vi "MB_Master Comm Tester.vi"() -> ()   [LabVIEW 2012]
doc: "Modbus Comm Tester\n\nThis VI demonstrates the usage of the Modbus Master API for both TCP and Serial connections.\nIt is also a useful tool for testing communication with your modbus device. You can test different\ncommunication parameters and coil/register address ranges without having to write any code.\n\nCopyright (c) 2016, Plasmionique Inc.\nAll rights reserved.\n\nLicense: BSD (2-Clause) - http://opensource.org/licenses/BSD-2-Clause"
uses:
  MB_Master/MB_Master.lvclass
  MB_ADU/MB_ADU.lvclass/MB_ADU.ctl
  MB_ADU/Read TX Data.vi
  MB_ADU/Read RX Data.vi
  MB_ADU/Read RX Timestamp.vi
  MB_Master_Serial/MB_Master_Serial.lvclass
  MB Master.lvlib
  MB_ADU/MB_ADU.lvclass
  MB_Master_TCP/MB_Master_TCP.lvclass
panel:
  in  "Poll Period (ms)":i32=100
  in  "Tab Control":enum32{"Page 1", "Page 2"}(tab)
  in  "Retries":i32=1
  in  "Timeout (ms)":u32=300
  in  "Flow Control":u16(ring) items=["None", "XON/XOFF", "RTS/CTS", "XON/XOFF & RTS/CTS", "DTR/DSR", "XON/XOFF & DTR/DSR"]
  in  "Parity":u16(ring) items=["None", "Odd", "Even", "Mark", "Space"]
  in  "Stop Bits":u16(ring)=10 items=["1.0"=10, "1.5"=15, "2.0"=20]
  in  "Baud Rate (bps)":u32(ring)=19200 items=["9600"=9600, "19200"=19200, "38400"=38400, "57600"=57600, "115200"=115200, "460800"=460800, "921600"=921600]
  in  "Slave Address":u8=1
  in  "Mode":enum16{"RTU", "ASCII"}(ring)
  in  "COM Port":refnum<visa-resource-name>
  in  "TCP_Port":u16=502 caption="Port"
  in  "IP Address":string="localhost"
  in  "TCP_Timeout":i32=10000 caption="Timeout (ms)"
  in  "TCP_Slave ID":u8=255 caption="Slave ID" format="%.0x"
  in  "Type":enum16{"Serial", "TCP"}(ring) caption="Connection Type"
  out "dt (ms)":u32
  in  "DI Poll":bool
  in  "IR Poll":bool
  in  "Exit":bool
  out "Last Error Time":string
  out "Last RX Time":string
  in  "Write Hld Regs":bool
  in  "Read Hld Regs":bool
  in  "HR QTY":u16=1 caption="Quantity"
  in  "HR SA":u16 caption="Starting Address" format="%.0x"
  in  "Holding Registers":u16[](array[numeric])
  in  "Read In Regs":bool
  in  "IR QTY":u16=1 caption="Quantity"
  in  "IR SA":u16 caption="Starting Address" format="%.0x"
  out "Input Registers":u16[](array[numeric])
  in  "Read DIs":bool
  in  "DI QTY":u16=1 caption="Quantity"
  in  "DI SA":u16 caption="Starting Address" format="%.0x"
  out "Discrete Inputs":bool[](array[boolean])
  in  "Write Coils":bool
  in  "Read Coils":bool
  in  "Coil QTY":u16=1 caption="Quantity"
  in  "Coil SA":u16 caption="Starting Address" format="%.0x"
  in  "Coils":bool[](array[boolean])
  out "Last TX":string
  out "Last RX":string
  out "Last Error Status":errorcluster
  out "Open?":bool
  in  "Close":bool
  in  "Open":bool
  # "Input Registers"
  # "Discrete Inputs"
  # "Communication Settngs"
  # "Communication Status"
  # "Holding Registers"
  # "Coils"
  # "See block diagram for description and usage notes."
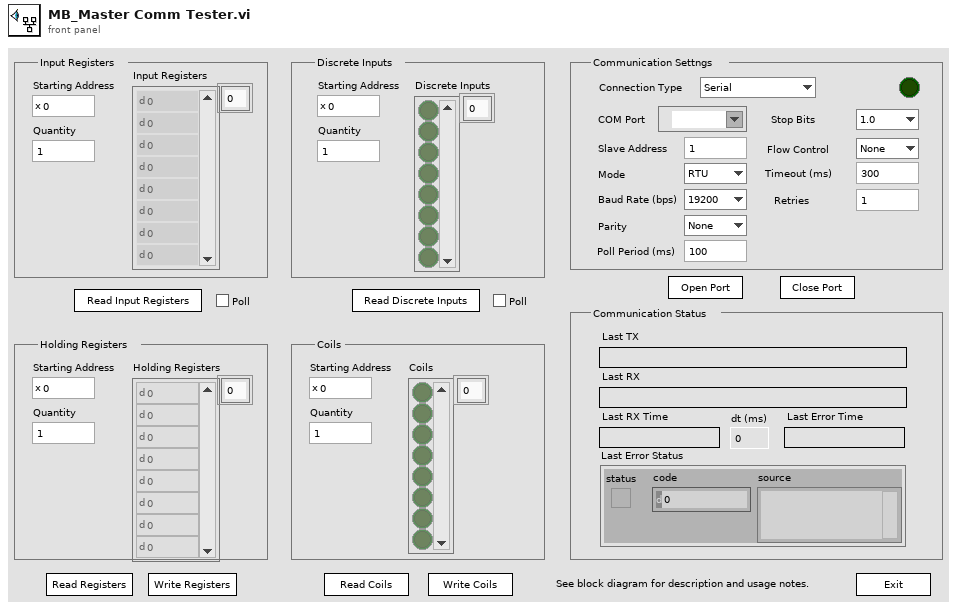
[diagram p1: front panel]
types:
  T1 = cluster{"baud rate (bps)":u32, "stop bits":u16, "parity":u16, "flow control":u16, "timeout":u32, "retries":i32}
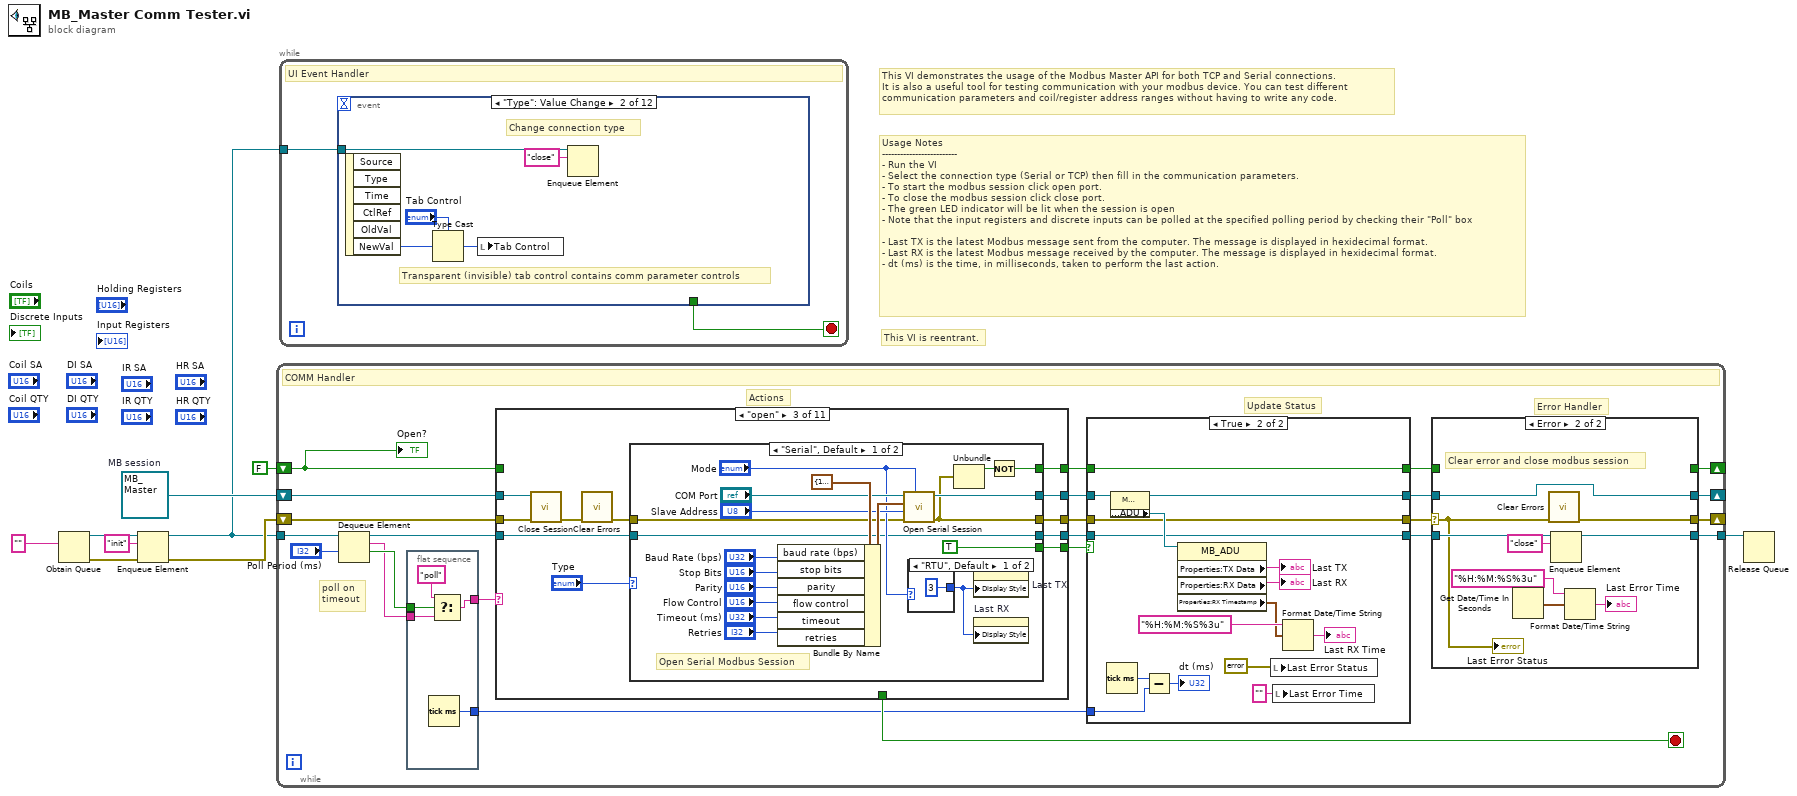
[diagram p0: block diagram]
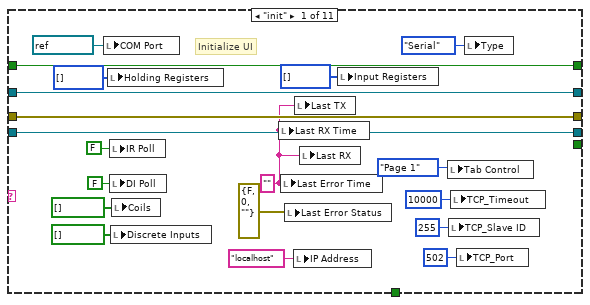
[diagram p4: hidden frame]
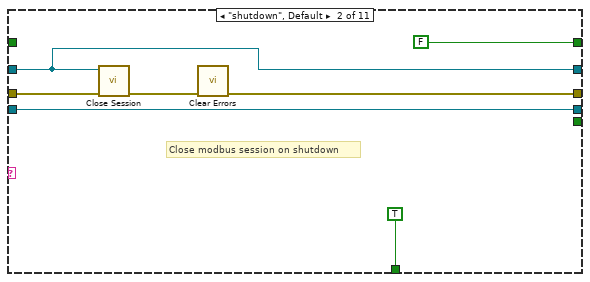
[diagram p5: hidden frame]
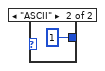
[diagram p6: hidden frame]
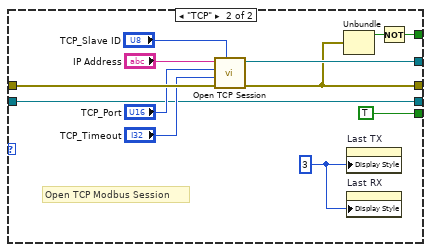
[diagram p7: hidden frame]
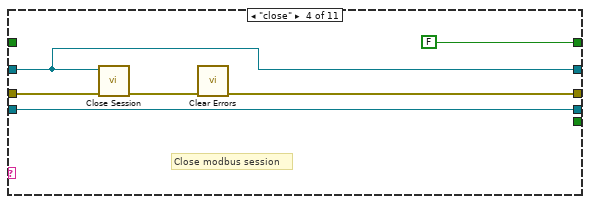
[diagram p8: hidden frame]
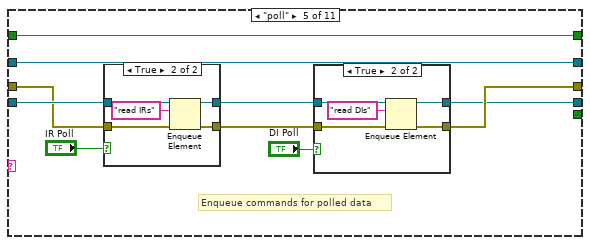
[diagram p9: hidden frame]
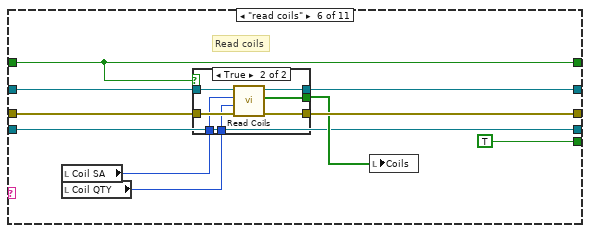
[diagram p12: hidden frame]
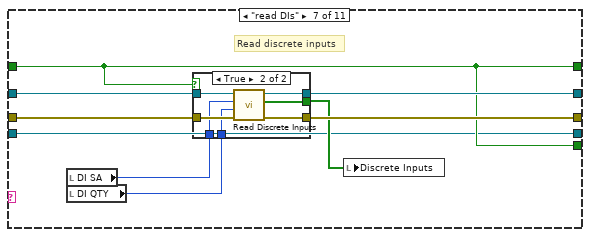
[diagram p14: hidden frame]
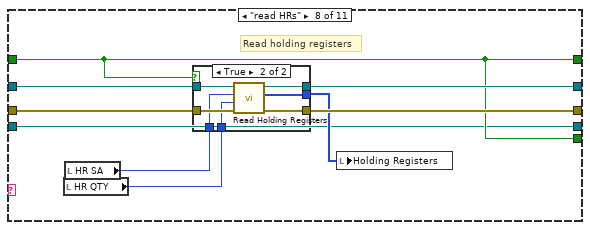
[diagram p16: hidden frame]
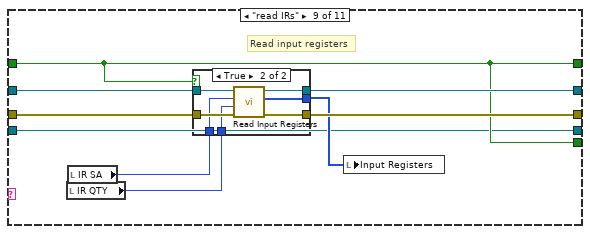
[diagram p18: hidden frame]
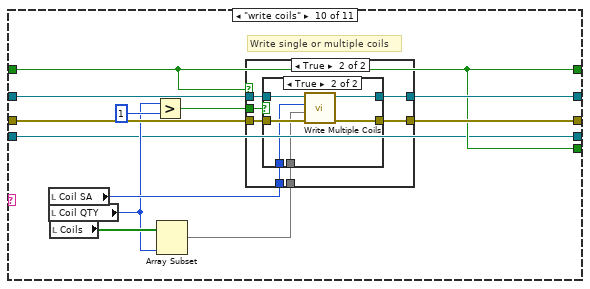
[diagram p20: hidden frame]
diagram:
  w7 = refnum<class "MB_Master.lvclass"> refnum  # MB session
  # "This VI is reentrant."
  # "Usage Notes\n-------------------------\n- Run the VI\n- Select the connection type (Serial or TCP) then fill in the communication parameters.\n- To start the modbus session click open port.\n- To close the modbus session click close port.\n- The green LED indicator will be lit when the session is open\n- Note that the input registers and discrete inputs can be polled at the specified polling period by checking their \"Poll\" box\n\n- Last TX is the latest Modbus message sent from the computer. The message is displayed in hexidecimal format.\n- Last RX is the latest Modbus message received by the computer. The message is displayed in hexidecimal format. \n- dt (ms) is the time, in milliseconds, taken to perform the last action."
  # "This VI demonstrates the usage of the Modbus Master API for both TCP and Serial connections.\nIt is also a useful tool for testing communication with your modbus device. You can test different\ncommunication parameters and coil/register address ranges without having to write any code."
  n1 = Obtain Queue(element data type="") -> (queue out=w6:refnum<queue>, error out=w4:errorcluster)  [unwired: 4 in, 1 out]
  n2 = Enqueue Element(queue=w6, element="init", error in (no error)=w4) -> (queue out=w2:refnum<queue>, error out=w3:errorcluster)  [unwired: 1 in, 1 out]
  n3 = while {
    tunnel: w2 -> [w33]
    shift-right: [w16] -> _
    shift-left: w7 -> [w32]
    shift-right: [w23] -> _
    shift-left: w3 -> [w24]
    shift-right: [w18] -> _
    shift-left: FALSE -> [w28]
    tunnel: [w22] -> w1
    stop <- w31 stop-if-true
    # "poll on\ntimeout"
    # "Actions"
    # "Error Handler"
    # "Update Status"
    # "COMM Handler"
    n4 = Dequeue Element(queue=w33, timeout in ms (-1)="Poll Period (ms)") -> (queue out=w30:refnum<queue>, element=w20:string, timed out?=w21:bool)  [unwired: 1 in, 1 out]
    n5 = flat-sequence {
      tunnel: [w51] -> w25
      tunnel: w21 -> [w50]
      tunnel: w20 -> [w49]
      tunnel: [w47] -> w19
      frame #0 {
        n6 = Tick Count (ms)() -> (millisecond timer value=w51:u32)
        n7 = Select(t="poll", s=w50, f=w49) -> (s? t:f=w47:string)
      }
    }
    n8 = case shown="\"open\"" w19 {
      tunnel: [w89 w94 w108 w144 w149 w179 w197 w215 w233 w253 w287] -> w29
      tunnel: w32 -> [w89 w94 w103 w144 w149 w181 w199 w217 w235 w256 w290]
      tunnel: [w88 w95 w107 w145 w151 w178 w196 w214 w232 w251 w285] -> w13
      tunnel: w24 -> [w88 w97 w102 w147 w154 w180 w198 w216 w234 w252 w286]
      tunnel: [_ TRUE _ _ _ _ _ _ _ _ _] -> w31
      tunnel: w30 -> [w79 w91 w99 w142 w156 w172 w191 w209 w227 w245 w279]
      tunnel: w28 -> [w86 _ _ _ w150 w176 w192 w210 w228 w246 w280]
      tunnel: [w86 FALSE w106 FALSE w150 w176 w192 w210 w228 w246 w280] -> w15
      tunnel: [_ _ w105 _ _ TRUE w192 w210 w228 w246 w280] -> w27
      tunnel: [w79 w91 w98 w142 w148 w172 w191 w209 w227 w245 w279] -> w11
      frame "init" {
        w87 = "" ("Last Error Time")
        # "Initialize UI"
        n9 = local write "COM Port"(refnum<visa-resource-name> refnum ("COM Port")) -> ()
        n10 = local write "Holding Registers"(u16[] [] ("Holding Registers")) -> ()
        n11 = local write "IR Poll"(FALSE ("IR Poll")) -> ()
        n12 = local write "DI Poll"(FALSE ("DI Poll")) -> ()
        n13 = local write "Discrete Inputs"(bool[] [] ("Coils")) -> ()
        n14 = local write "Coils"(bool[] [] ("Coils")) -> ()
        n15 = local write "Last RX Time"(w87) -> ()
        n16 = local write "Last Error Time"(w87) -> ()
        n17 = local write "Last Error Status"(errorcluster {"status"=FALSE, "code"=0, "source"=""} ("Last Error Status")) -> ()
        n18 = local write "IP Address"("localhost" ("IP Address")) -> ()
        n19 = local write "Last TX"(w87) -> ()
        n20 = local write "Last RX"(w87) -> ()
        n21 = local write "Input Registers"(u16[] [] ("Input Registers")) -> ()
        n22 = local write "Tab Control"(enum32{"Page 1", "Page 2"}."Page 1" ("Tab Control")) -> ()
        n23 = local write "TCP_Slave ID"(u8 255 ("TCP_Slave ID")) -> ()
        n24 = local write "TCP_Timeout"(10000 ("TCP_Timeout")) -> ()
        n25 = local write "TCP_Port"(u16 502 ("TCP_Port")) -> ()
        n26 = local write "Type"(enum16{"Serial", "TCP"}."Serial" ("Type")) -> ()
      }
      frame "shutdown", Default {
        # "Close modbus session on shutdown"
        n27 = call-dynamic "Close Session.vi"("error in (no error)"=w97, "MB session in"=w94) -> ("error out"=w96:errorcluster)  [unwired: 9 in]
        n28 = call <vilib>:"Clear Errors.vi"("error in (no error)"=w96) -> ("error out"=w95:errorcluster)  [unwired: 6 in]
      }
      frame "open" {
        n29 = call-dynamic "Close Session.vi"("error in (no error)"=w102, "MB session in"=w103) -> ("error out"=w104:errorcluster)  [unwired: 9 in]
        n30 = call <vilib>:"Clear Errors.vi"("error in (no error)"=w104) -> ("error out"=w101:errorcluster)  [unwired: 6 in]
        n31 = case shown="\"Serial\", Default" "Type" {
          tunnel: [w117 w132] -> w108
          tunnel: [w116 w130] -> w107
          tunnel: [w114 w134] -> w106
          tunnel: [TRUE TRUE] -> w105
          tunnel: w101 -> [w110 w141]
          tunnel: [w109 w136] -> w98
          tunnel: w99 -> [w109 w136]
          frame "Serial", Default {
            # "Open Serial Modbus Session"
            n32 = Bundle By Name(cluster=T1 {"baud rate (bps)"=19200, "stop bits"=10, "parity"=0, "flow control"=0, "timeout"=1000, "retries"=1} ("Serial Config"), "baud rate (bps)"="Baud Rate (bps)", "stop bits"="Stop Bits", "parity"="Parity", "flow control"="Flow Control", "timeout"="Timeout (ms)", "retries"="Retries") -> (w119:T1)
            n33 = call "Open Serial Session.vi"("Mode (RTU)"="Mode", "Error in"=w110, "Slave ID"="Slave Address", "Serial Config"=w119, "VISA Resource"="COM Port") -> ("Error out"=w116:errorcluster, "MB_Serial session"=w117:refnum<class "MB_Master_Serial.lvclass">)  [unwired: 5 in]
            n34 = case shown="\"RTU\", Default" "Mode" {
              tunnel: [u32 3 ("Display Style") u32 1 ("Display Style")] -> w111
              frame "RTU", Default {
              }
              frame "ASCII" {
              }
            }
            n35 = Unbundle(w116) -> ("status"=w115:bool)  [unwired: 2 out]
            n36 = property on="Last TX" class="Str"("Display Style"=w111) -> ()  [unwired: 2 in, 2 out]
            n37 = property on="Last RX" class="Str"("Display Style"=w111) -> ()  [unwired: 2 in, 2 out]
            n38 = Not(x=w115) -> (.not. x?=w114:bool)
          }
          frame "TCP" {
            w133 = u32 3 ("Display Style")
            # "Open TCP Modbus Session"
            n39 = call "Open TCP Session.vi"("Slave ID (255)"="TCP_Slave ID", "error in (no error)"=w141, "Timeout (10000)"="TCP_Timeout", "Port (502)"="TCP_Port", "IP Address"="IP Address") -> ("error out"=w130:errorcluster, "MB_TCP session"=w132:refnum<class "MB_Master_TCP.lvclass">)  [unwired: 5 in]
            n40 = Unbundle(w130) -> ("status"=w135:bool)  [unwired: 2 out]
            n41 = property on="Last TX" class="Str"("Display Style"=w133) -> ()  [unwired: 2 in, 2 out]
            n42 = property on="Last RX" class="Str"("Display Style"=w133) -> ()  [unwired: 2 in, 2 out]
            n43 = Not(x=w135) -> (.not. x?=w134:bool)
          }
        }
      }
      frame "close" {
        # "Close modbus session"
        n44 = call-dynamic "Close Session.vi"("error in (no error)"=w147, "MB session in"=w144) -> ("error out"=w146:errorcluster)  [unwired: 9 in]
        n45 = call <vilib>:"Clear Errors.vi"("error in (no error)"=w146) -> ("error out"=w145:errorcluster)  [unwired: 6 in]
      }
      frame "poll" {
        # "Enqueue commands for polled data"
        n46 = case shown="True" "IR Poll" {
          tunnel: w156 -> [w166 w170]
          tunnel: [w166 w169] -> w155
          tunnel: w154 -> [w165 w168]
          tunnel: [w165 w167] -> w152
          frame False {
          }
          frame True {
            n47 = Enqueue Element(queue=w170, element="read IRs", error in (no error)=w168) -> (queue out=w169:refnum<queue>, error out=w167:errorcluster)  [unwired: 1 in, 1 out]
          }
        }
        n48 = case shown="True" "DI Poll" {
          tunnel: w155 -> [w158 w163]
          tunnel: w152 -> [w159 w162]
          tunnel: [w159 w161] -> w151
          tunnel: [w158 w160] -> w148
          frame False {
          }
          frame True {
            n49 = Enqueue Element(queue=w163, element="read DIs", error in (no error)=w162) -> (queue out=w160:refnum<queue>, error out=w161:errorcluster)  [unwired: 1 in, 1 out]
          }
        }
      }
      frame "read coils" {
        # "Read coils"
        n50 = local read "Coil SA"() -> (w175:u16)
        n51 = local read "Coil QTY"() -> (w174:u16)
        n52 = case shown="True" w176 {
          tunnel: w181 -> [w183 w190]
          tunnel: w180 -> [w182 w189]
          tunnel: [w183 w188] -> w179
          tunnel: [w182 w187] -> w178
          tunnel: w175 -> [_ w186]
          tunnel: w174 -> [_ w185]
          tunnel: [_ w184] -> w177
          frame False {
          }
          frame True {
            n53 = call "Read Coils.vi"("error in (no error)"=w189, "quantity"=w185, "starting address"=w186, "MB session in"=w190) -> ("error out"=w187:errorcluster, "Coils"=w184:bool[], "MB session out"=w188:refnum<class "MB_Master.lvclass">)  [unwired: 5 in]
          }
        }
        n54 = local write "Coils"(w177) -> ()
      }
      frame "read DIs" {
        # "Read discrete inputs"
        n55 = local read "DI SA"() -> (w194:u16)
        n56 = local read "DI QTY"() -> (w193:u16)
        n57 = case shown="True" w192 {
          tunnel: w199 -> [w201 w208]
          tunnel: w198 -> [w200 w207]
          tunnel: [w201 w206] -> w197
          tunnel: [w200 w205] -> w196
          tunnel: w194 -> [_ w204]
          tunnel: w193 -> [_ w203]
          tunnel: [_ w202] -> w195
          frame False {
          }
          frame True {
            n58 = call "Read Discrete Inputs.vi"("error in (no error)"=w207, "quantity"=w203, "starting address"=w204, "MB session in"=w208) -> ("error out"=w205:errorcluster, "Inputs"=w202:bool[], "MB session out"=w206:refnum<class "MB_Master.lvclass">)  [unwired: 5 in]
          }
        }
        n59 = local write "Discrete Inputs"(w195) -> ()
      }
      frame "read HRs" {
        # "Read holding registers"
        n60 = local read "HR QTY"() -> (w211:u16)
        n61 = local read "HR SA"() -> (w212:u16)
        n62 = case shown="True" w210 {
          tunnel: w217 -> [w219 w226]
          tunnel: w216 -> [w218 w225]
          tunnel: [w219 w224] -> w215
          tunnel: [w218 w223] -> w214
          tunnel: w212 -> [_ w222]
          tunnel: w211 -> [_ w221]
          tunnel: [_ w220] -> w213
          frame False {
          }
          frame True {
            n63 = call "Read Holding Registers.vi"("error in (no error)"=w225, "quantity"=w221, "starting address"=w222, "MB session in"=w226) -> ("error out"=w223:errorcluster, "Registers"=w220:u16[], "MB session out"=w224:refnum<class "MB_Master.lvclass">)  [unwired: 5 in]
          }
        }
        n64 = local write "Holding Registers"(w213) -> ()
      }
      frame "read IRs" {
        # "Read input registers"
        n65 = local read "IR QTY"() -> (w229:u16)
        n66 = local read "IR SA"() -> (w230:u16)
        n67 = case shown="True" w228 {
          tunnel: w235 -> [w237 w244]
          tunnel: w234 -> [w236 w243]
          tunnel: [w237 w242] -> w233
          tunnel: [w236 w241] -> w232
          tunnel: w230 -> [_ w240]
          tunnel: w229 -> [_ w239]
          tunnel: [_ w238] -> w231
          frame False {
          }
          frame True {
            n68 = call "Read Input Registers.vi"("error in (no error)"=w243, "quantity"=w239, "starting address"=w240, "MB session in"=w244) -> ("error out"=w241:errorcluster, "Registers"=w238:u16[], "MB session out"=w242:refnum<class "MB_Master.lvclass">)  [unwired: 5 in]
          }
        }
        n69 = local write "Input Registers"(w231) -> ()
      }
      frame "write coils" {
        # "Write single or multiple coils"
        n70 = local read "Coil SA"() -> (w250:u16)
        n71 = local read "Coil QTY"() -> (w248:u16)
        n72 = local read "Coils"() -> (w249:bool[])
        n73 = Greater?(x=w248, y=u16 1) -> (0:w254:bool)
        n74 = Array Subset(array=w249, length=w248) -> (w247:bool[])  [unwired: 1 in]
        n75 = case shown="True" w246 {
          tunnel: w256 -> [w258 w265]
          tunnel: w254 -> [_ w264]
          tunnel: [w258 w263] -> w253
          tunnel: w252 -> [w257 w262]
          tunnel: [w257 w261] -> w251
          tunnel: w250 -> [_ w260]
          tunnel: w247 -> [_ w259]
          frame False {
          }
          frame True {
            n76 = case shown="True" w264 {
              tunnel: w265 -> [w272 w278]
              tunnel: [w266 w277] -> w263
              tunnel: w262 -> [w271 w276]
              tunnel: [w267 w275] -> w261
              tunnel: w260 -> [w270 w274]
              tunnel: w259 -> [w269 w273]
              frame False {
                n77 = Index Array(array=w269) -> (element=w268:bool)  [unwired: 1 in]
                n78 = call "Write Single Coil.vi"("error in (no error)"=w271, "value"=w268, "address"=w270, "MB session in"=w272) -> ("error out"=w267:errorcluster, "MB session out"=w266:refnum<class "MB_Master.lvclass">)  [unwired: 6 in]
              }
              frame True {
                n79 = call "Write Multiple Coils.vi"("error in (no error)"=w276, "values"=w273, "starting address"=w274, "MB session in"=w278) -> ("error out"=w275:errorcluster, "MB session out"=w277:refnum<class "MB_Master.lvclass">)  [unwired: 6 in]
              }
            }
          }
        }
      }
      frame "write HRs" {
        # "Write single or multiple holding registers"
        n80 = local read "Holding Registers"() -> (w283:u16[])
        n81 = local read "HR QTY"() -> (w282:u16)
        n82 = local read "HR SA"() -> (w284:u16)
        n83 = Greater?(x=w282, y=u16 1) -> (0:w288:bool)
        n84 = Array Subset(array=w283, length=w282) -> (w281:u16[])  [unwired: 1 in]
        n85 = case shown="True" w280 {
          tunnel: w290 -> [w292 w299]
          tunnel: w288 -> [_ w298]
          tunnel: [w292 w297] -> w287
          tunnel: w286 -> [w291 w296]
          tunnel: [w291 w295] -> w285
          tunnel: w284 -> [_ w294]
          tunnel: w281 -> [_ w293]
          frame False {
          }
          frame True {
            n86 = case shown="True" w298 {
              tunnel: w299 -> [w306 w312]
              tunnel: [w300 w311] -> w297
              tunnel: w296 -> [w305 w310]
              tunnel: [w301 w309] -> w295
              tunnel: w294 -> [w304 w308]
              tunnel: w293 -> [w303 w307]
              frame False {
                n87 = Index Array(array=w303) -> (element=w302:u16)  [unwired: 1 in]
                n88 = call "Write Single Register.vi"("error in (no error)"=w305, "value"=w302, "address"=w304, "MB session in"=w306) -> ("error out"=w301:errorcluster, "MB session out"=w300:refnum<class "MB_Master.lvclass">)  [unwired: 6 in]
              }
              frame True {
                n89 = call "Write Multiple Registers.vi"("error in (no error)"=w310, "values"=w307, "starting address"=w308, "MB session in"=w312) -> ("error out"=w309:errorcluster, "MB session out"=w311:refnum<class "MB_Master.lvclass">)  [unwired: 6 in]
              }
            }
          }
        }
      }
    }
    n90 = case shown="True" w27 {
      tunnel: w29 -> [w55 w56]
      tunnel: [w55 w69] -> w17
      tunnel: w25 -> [_ w63]
      tunnel: w15 -> [w54 w59]
      tunnel: [w54 w59] -> w14
      tunnel: w13 -> [w53 w58]
      tunnel: [w53 w58] -> w12
      tunnel: w11 -> [w52 w57]
      tunnel: [w52 w57] -> w10
      frame False {
      }
      frame True {
        n91 = Tick Count (ms)() -> (millisecond timer value=w62:u32)
        n92 = property class="MB_Master"(reference=w56) -> (reference out=w69:refnum<class "MB_Master.lvclass">, "Properties:ADU"=w70:refnum<class "MB_ADU.lvclass">)  [unwired: 1 in, 1 out]
        n93 = Subtract(x=w62, y=w63) -> (x-y=→"dt (ms)":u32)
        n94 = property class="MB_ADU"(reference=w70) -> ("Properties:TX Data"=→"Last TX":string, "Properties:RX Data"=→"Last RX":string, "Properties:RX Timestamp"=w60:timestamp)  [unwired: 1 in, 2 out]
        n95 = local write "Last Error Status"(errorcluster {"status"=FALSE, "code"=0, "source"=""} ("Last Error Status")) -> ()
        n96 = local write "Last Error Time"("" ("Last Error Time")) -> ()
        n97 = Format Date/Time String(time format string (%c)="%H:%M:%S%3u", seconds (now)=w60) -> (date/time string=→"Last RX Time":string)  [unwired: 1 in]
      }
    }
    n98 = case shown="Error" w12 {
      selector: w12 -> [w37 w39]
      tunnel: [w37 w43] -> w23
      tunnel: w10 -> [w36 w41]
      tunnel: [w36 w40] -> w22
      tunnel: w14 -> [w35 _]
      tunnel: [w35 _] -> w18
      tunnel: w17 -> [w34 w38]
      tunnel: [w34 w38] -> w16
      frame No Error {
      }
      frame Error {
        # "Clear error and close modbus session"
        n99 = Get Date/Time In Seconds() -> (seconds since 1Jan1904=w44:timestamp)
        n100 = call <vilib>:"Clear Errors.vi"("error in (no error)"=w39) -> ("error out"=w43:errorcluster)  [unwired: 6 in]
        n101 = Enqueue Element(queue=w41, element="close") -> (queue out=w40:refnum<queue>)  [unwired: 2 in, 2 out]
        n102 = Format Date/Time String(time format string (%c)="%H:%M:%S%3u", seconds (now)=w44) -> (date/time string=→"Last Error Time":string)  [unwired: 1 in]
        "Last Error Status" <- w39
      }
    }
    "Open?" <- w28
  }
  n103 = while {
    tunnel: w2 -> [w314]
    stop <- w313 stop-if-true
    # "UI Event Handler"
    n104 = event shown="[1] \"Type\": Value Change" {
      selector: _ -> [_ _ _ _ _ _ _ _ _ _ _ _]
      dyn-events: _ -> [_ _ _ _ _ _ _ _ _ _ _ _]
      timeout: _ -> [_ _ _ _ _ _ _ _ _ _ _ _]
      tunnel: w314 -> [_ w318 w321 w322 w324 w326 w328 w330 w332 w334 w336 w340]
      tunnel: [_ _ _ _ _ _ _ _ _ _ TRUE TRUE] -> w313
      event Timeout {
        n105 = event-data() -> ()  [unwired: 1 in, 3 out]
      }
      event "Type": Value Change {
        # "Transparent (invisible) tab control contains comm parameter controls"
        # "Change connection type"
        n106 = event-data() -> ("NewVal"=w317:enum16{"Serial", "TCP"})  [unwired: 1 in, 5 out]
        n107 = Type Cast(type="Tab Control", x=w317) -> (*(type *) &x=w315:enum32{"Page 1", "Page 2"})
        n108 = local write "Tab Control"(w315) -> ()
        n109 = Enqueue Element(queue=w318, element="close") -> ()  [unwired: 2 in, 3 out]
      }
      event "Open": Value Change {
        # "Open modbus session"
        n110 = event-data() -> ()  [unwired: 1 in, 6 out]
        n111 = Enqueue Element(queue=w321, element="open") -> ()  [unwired: 2 in, 3 out]
      }
      event "Close": Value Change {
        # "Close modbus session"
        n112 = event-data() -> ()  [unwired: 1 in, 6 out]
        n113 = Enqueue Element(queue=w322, element="close") -> ()  [unwired: 2 in, 3 out]
      }
      event "Read Coils": Value Change {
        n114 = event-data() -> ()  [unwired: 1 in, 6 out]
        n115 = Enqueue Element(queue=w324, element="read coils") -> ()  [unwired: 2 in, 3 out]
      }
      event "Read DIs": Value Change {
        n116 = event-data() -> ()  [unwired: 1 in, 6 out]
        n117 = Enqueue Element(queue=w326, element="read DIs") -> ()  [unwired: 2 in, 3 out]
      }
      event "Write Coils": Value Change {
        n118 = event-data() -> ()  [unwired: 1 in, 6 out]
        n119 = Enqueue Element(queue=w328, element="write coils") -> ()  [unwired: 2 in, 3 out]
      }
      event "Read In Regs": Value Change {
        n120 = event-data() -> ()  [unwired: 1 in, 6 out]
        n121 = Enqueue Element(queue=w330, element="read IRs") -> ()  [unwired: 2 in, 3 out]
      }
      event "Read Hld Regs": Value Change {
        n122 = event-data() -> ()  [unwired: 1 in, 6 out]
        n123 = Enqueue Element(queue=w332, element="read HRs") -> ()  [unwired: 2 in, 3 out]
      }
      event "Write Hld Regs": Value Change {
        n124 = event-data() -> ()  [unwired: 1 in, 6 out]
        n125 = Enqueue Element(queue=w334, element="write HRs") -> ()  [unwired: 2 in, 3 out]
      }
      event Panel Close? {
        n126 = event-data() -> ()  [unwired: 1 in, 4 out]
        n127 = Enqueue Element(queue=w336, element="shutdown") -> ()  [unwired: 2 in, 3 out]
        n128 = event-data("Discard?"=TRUE) -> ()  [unwired: 1 in, 1 out]
      }
      event "Exit": Value Change {
        n129 = event-data() -> ()  [unwired: 1 in, 6 out]
        n130 = Enqueue Element(queue=w340, element="shutdown") -> ()  [unwired: 2 in, 3 out]
      }
    }
  }
  n131 = Release Queue(queue=w1) -> ()  [unwired: 2 in, 3 out]
